vi "Read Connection Ind.vi"(8 "error in (no error)":errorcluster, 11 "Anritsu Call Box_Implement in":refnum<class "Anritsu Call Box_Implement.lvclass">) -> (0 "error out":errorcluster, 2 "Connection Ind":T1, 3 "Anritsu Call Box_Implement out":refnum<class "Anritsu Call Box_Implement.lvclass">)   [LabVIEW 2023, in "ANRITSU Call Box.lvlib" / "Anritsu Call Box_Implement.lvclass"]
uses:
  Anritsu Call Box_Implement.lvclass
  Anritsu Call Box_Implement.lvclass/Anritsu Call Box_Implement.ctl
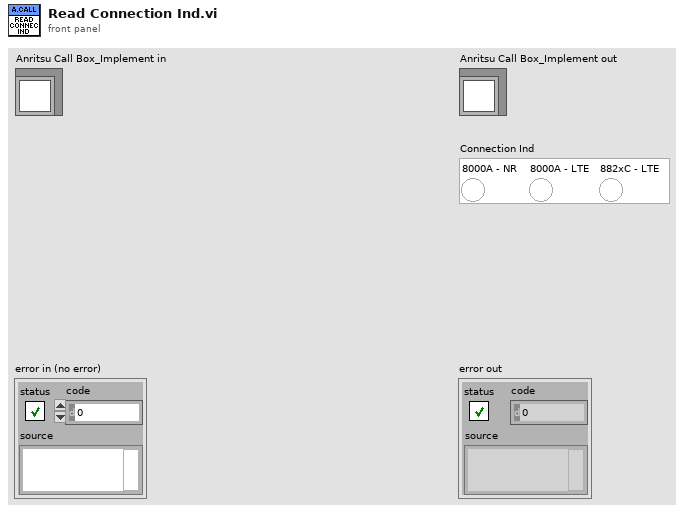
[diagram p1: front panel]
types:
  T1 = cluster{"8000A - NR":bool, "8000A - LTE":bool, "882xC - LTE":bool}
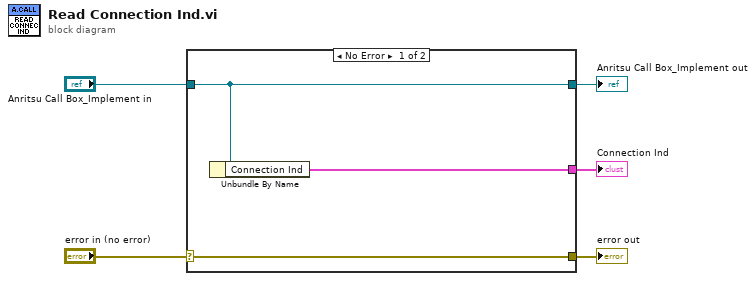
[diagram p0: block diagram]
diagram:
  n1 = case shown="No Error" "error in (no error)" {
    selector: "error in (no error)" -> [w8 w9]
    tunnel: [w8 w9] -> w4
    tunnel: [w7 w10] -> w2
    tunnel: "Anritsu Call Box_Implement in" -> [w7 w10]
    tunnel: [w6 _] -> w1
    frame No Error {
      n2 = Unbundle By Name(w7) -> ("Connection Ind"=w6:T1)
    }
    frame Error {
    }
  }
  "error out" <- w4
  "Anritsu Call Box_Implement out" <- w2
  "Connection Ind" <- w1
